vi "FuncVI-Mean.vi"(5 "InstanceRef":T2, 9 "arg list":T1[](array[typedef]) {"num" format="%.2f"}) -> (0 "error out":bool, 3 "result":T1 {"num" format="%.2f"})   [LabVIEW 2021]
doc: "::: CalcExpress Toolkit :::\nCopyright (c) 2000-2026 Konstantin Shifershteyn. All rights reserved."
uses:
  cetypes.llb/CalcExpress Function Argument Info.ctl
  cetypes.llb/CalcExpress Instance RefNum.ctl
  <vilib>/Analysis/baseanly.llb/Mean (DBL).vi
  <vilib>/Analysis/NI_AALBase.lvlib
panel:
  in  "max arg num":i32=1000
  in  "min arg num":i32=1
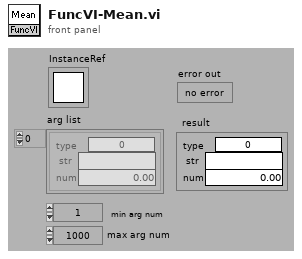
[diagram p1: front panel]
types:
  T1 = typedef "CalcExpress Function Argument Info.ctl" = cluster{"type":u32, "str":string, "num":dbl}
  T2 = typedef "CalcExpress Instance RefNum.ctl" = refnum<k1>
  T3 = enum32{"String", "DBL Number", "identifier", "1D Array of DBL", "2D Array of DBL", "CDB Number", "1D Array of CDB", "2D Array of CDB", "1D Array of String", "2D Array of String", "Unknown data type"}
  T4 = cluster{"use this constant to specify a predefined type":enum32{"String", "DBL Number", "identifier", "1D Array of DBL", "2D Array of DBL", "CDB Number", "1D Array of CDB", "2D Array of CDB", "1D Array of String", "2D Array of String", "Unknown data type"}, string, "mean":dbl}
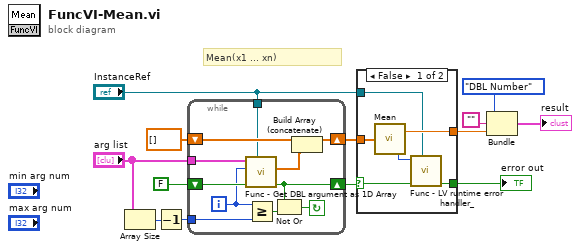
[diagram p0: block diagram]
diagram:
  # "Mean(x1 ... xn)"
  n1 = Array Size(array="arg list") -> (size(s)=w7:i32)
  n2 = Decrement(x=w7) -> (x-1=w1:i32)
  n3 = while {
    tunnel: "InstanceRef" -> [w15]
    tunnel: "arg list" -> [w16]
    shift-left: dbl[] [] -> [w18]
    shift-right: [w17] -> w5
    tunnel: w1 -> [w14]
    shift-left: FALSE ("error out") -> [w24]
    shift-right: [w21] -> w2
    i -> [w23]
    stop <- w20 continue-if-true
    n4 = call "Func - Get DBL argument as 1D Array.vi"("InstanceRef"=w15, "error in"=w24, "arg idx"=w23, "arg list"=w16) -> ("error out"=w21:bool, "1D data"=w19:dbl[])  [unwired: 4 in, 2 out]
    n5 = Greater Or Equal?(x=w23, y=w14) -> (x >= y?=w22:bool)
    n6 = Not Or(1:w22, 2:w21) -> (0:w20:bool)
    n7 = Build Array (concatenate)(w18, w19) -> (w17:dbl[])
  }
  n8 = case shown="False" w2 {
    selector: w2 -> [w29 w31]
    tunnel: w5 -> [w30 _]
    tunnel: [w27 _] -> w12
    tunnel: [w26 w31] -> w13
    tunnel: "InstanceRef" -> [w25 _]
    frame False {
      n9 = call-poly <vilib>:"Mean.vi"("X"=w30) -> ("mean"=w27:dbl, "error"=w28:i32)
      n10 = call "Func - LV runtime error handler_.vi"("InstanceRef"=w25, "error in"=w29, "LabVIEW error code"=w28) -> ("error out"=w26:bool)  [unwired: 8 in]
    }
    frame True {
    }
  }
  "error out" <- w13
  n11 = Bundle("use this constant to specify a predefined type"=T3."DBL Number", "", "mean"=w12) -> (→"result":T4)  [unwired: 1 in]
